vi "Generer_profil EPC3000.vi"(0 "Temps (s)":dbl[](array[numeric]) format="%#.1f", 1 "Num_Prog":u8, 2 "Températures (°C)":dbl[](array[numeric]) format="%#.1f", 3 "Evennements_entrée":T1, 4 "Programmes et config":T2 {"Programme 10"."Received Value" format="%#.1f"; "Programme 9"."Received Value" format="%#.1f"; "Programme 8"."Received Value" format="%#.1f"; "Programme 7"."Received Value" format="%#.1f"; "Programme 6"."Received Value" format="%#.1f"; "Programme 5"."Received Value" format="%#.1f"; "Configuration"."?" format="%#.1f"; "Programme 1"."Received Value" format="%#.1f"; "Programme 2"."Received Value" format="%#.1f"; "Programme 3"."Received Value" format="%#.1f"; "Programme 4"."Received Value" format="%#.1f"}) -> (5 "Temps (s)":dbl[](array[numeric]) format="%#.1f", 6 "Températures (°C)":dbl[](array[numeric]) format="%#.1f", 7 "Evennements_sortie":T1)   [LabVIEW 2022 SP3]
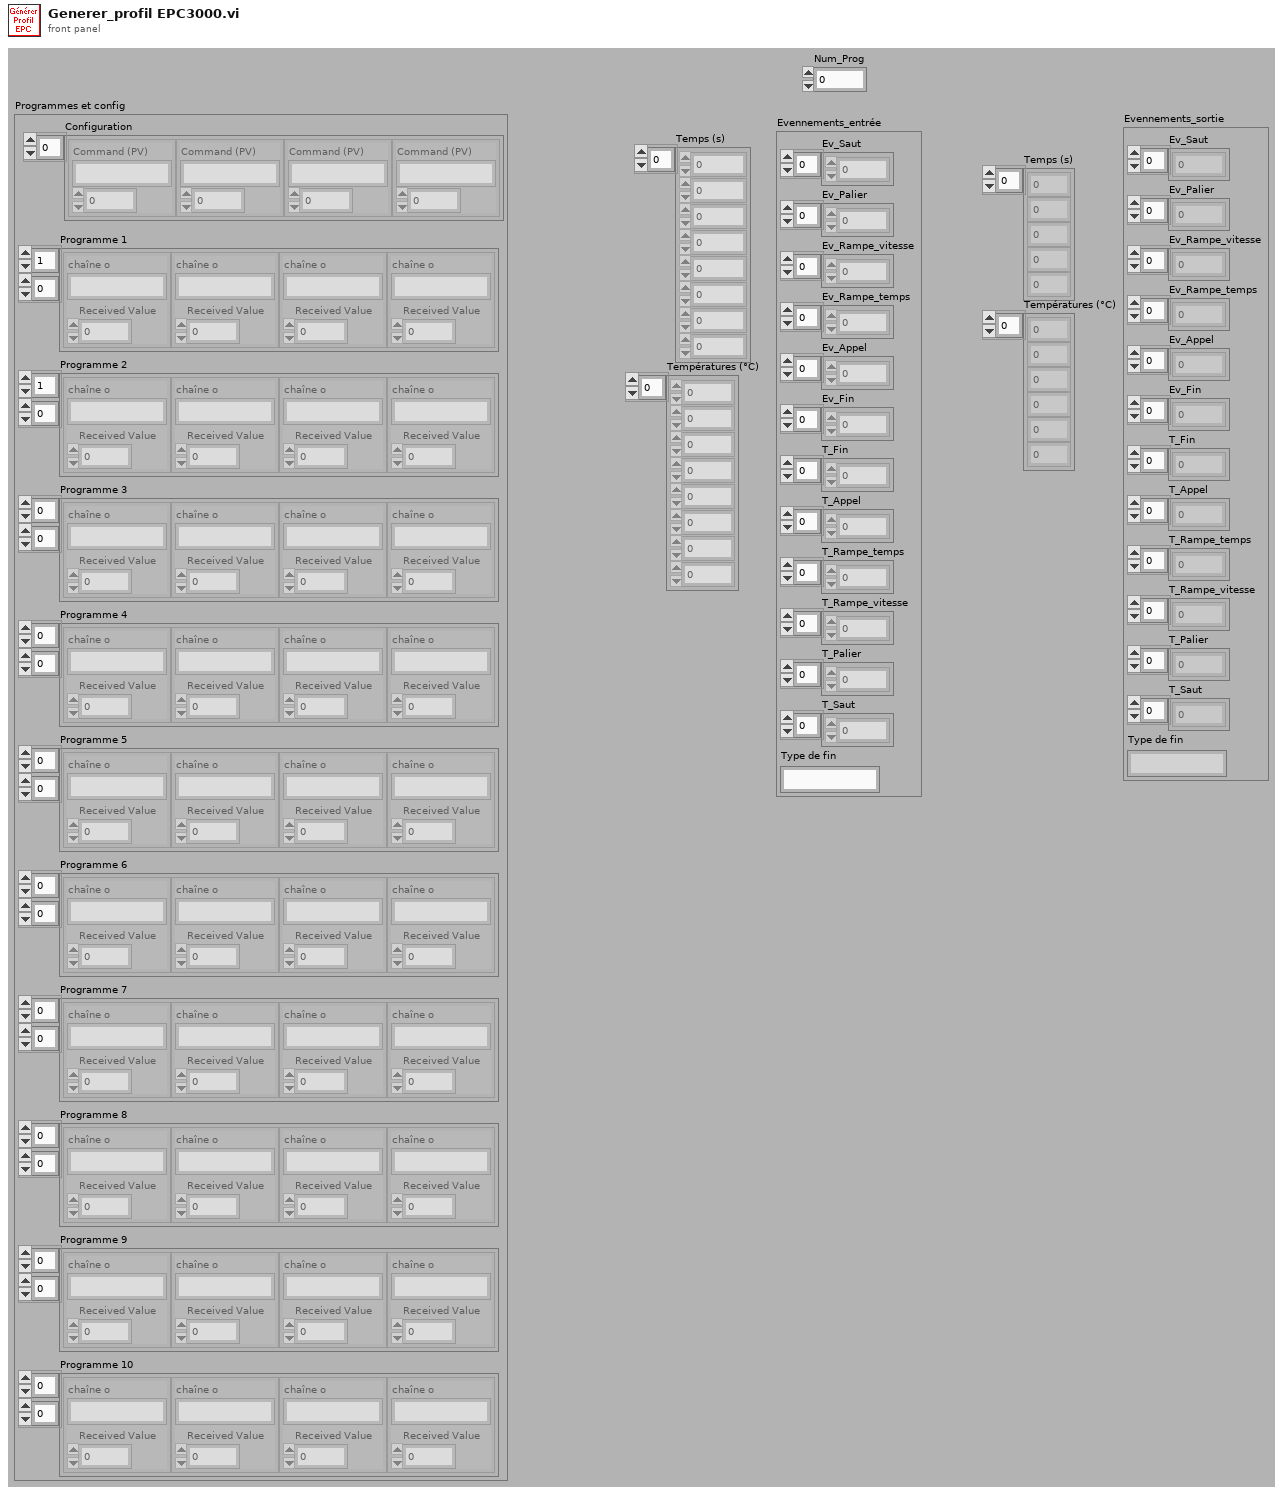
[diagram p1: front panel]
types:
  T1 = cluster{"Ev_Saut":dbl[], "Ev_Palier":dbl[], "Ev_Rampe_vitesse":dbl[], "Ev_Rampe_temps":dbl[], "Ev_Appel":dbl[], "Ev_Fin":dbl[], "T_Fin":dbl[], "T_Appel":dbl[], "T_Rampe_temps":dbl[], "T_Rampe_vitesse":dbl[], "T_Palier":dbl[], "T_Saut":dbl[], "Type de fin":string}
  T2 = cluster{"Configuration":cluster{"Command (PV)":string, dbl}[], "Programme 1":cluster{"chaîne o":string, "Received Value":dbl}[][], "Programme 2":cluster{"chaîne o":string, "Received Value":dbl}[][], "Programme 3":cluster{"chaîne o":string, "Received Value":dbl}[][], "Programme 4":cluster{"chaîne o":string, "Received Value":dbl}[][], "Programme 5":cluster{"chaîne o":string, "Received Value":dbl}[][], "Programme 6":cluster{"chaîne o":string, "Received Value":dbl}[][], "Programme 7":cluster{"chaîne o":string, "Received Value":dbl}[][], "Programme 8":cluster{"chaîne o":string, "Received Value":dbl}[][], "Programme 9":cluster{"chaîne o":string, "Received Value":dbl}[][], "Programme 10":cluster{"chaîne o":string, "Received Value":dbl}[][]}
  T3 = cluster{"chaîne o":string, "Received Value":dbl}[][]
  T4 = cluster{"chaîne o":string, "Received Value":dbl}[]
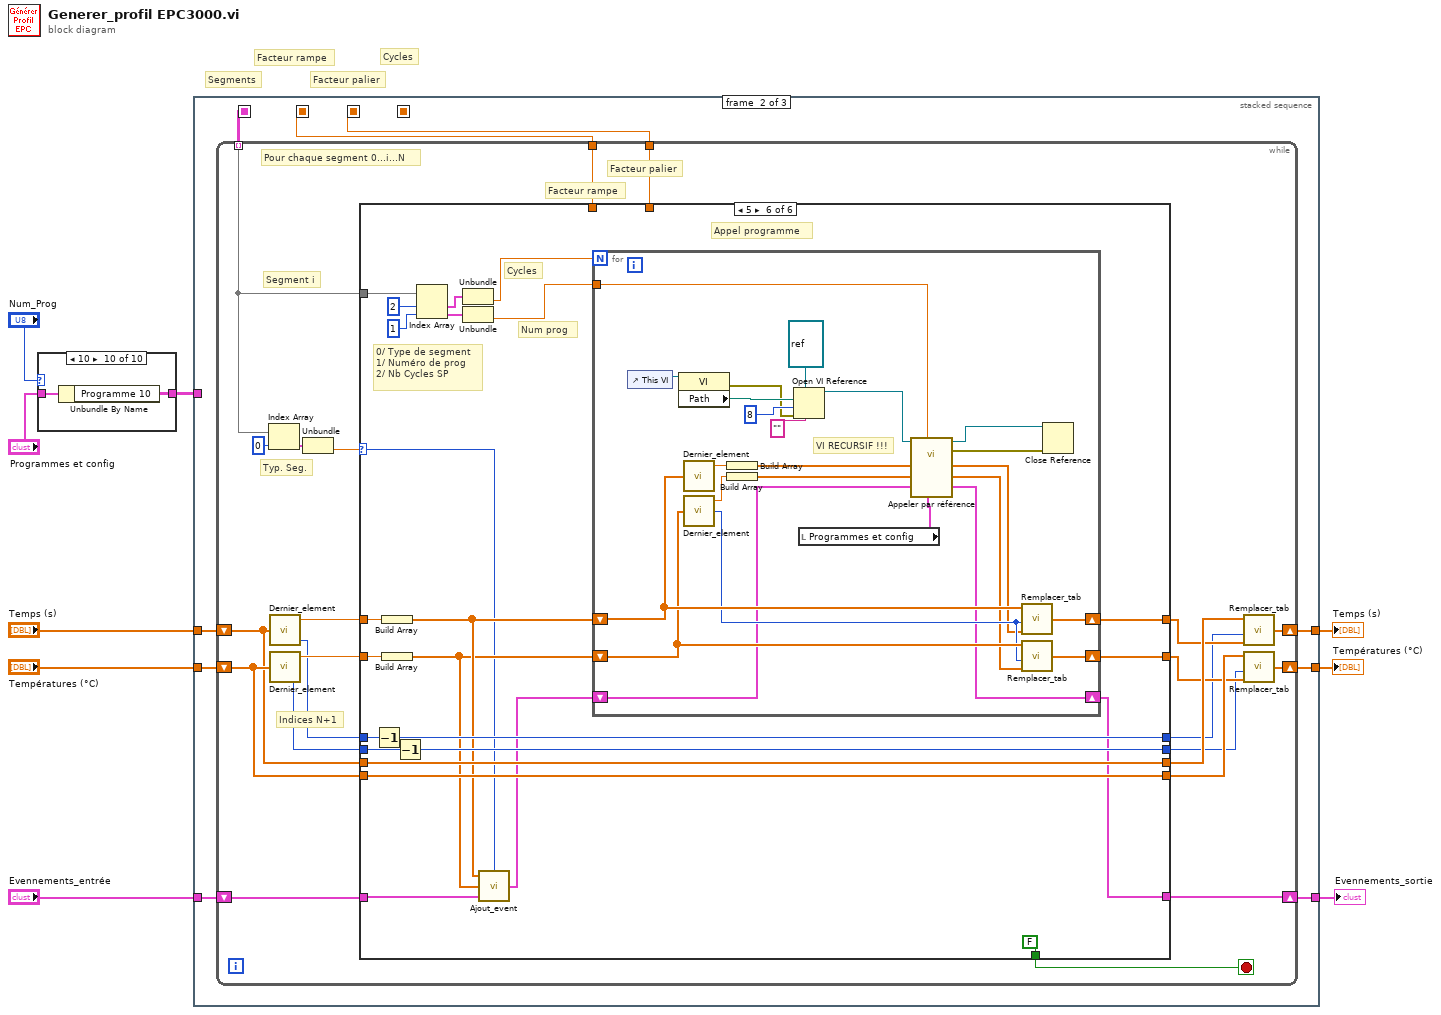
[diagram p0: block diagram]
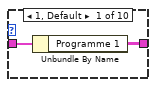
[diagram p2: hidden frame]
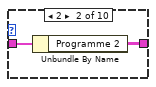
[diagram p3: hidden frame]
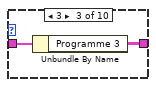
[diagram p4: hidden frame]
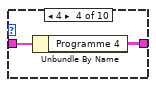
[diagram p5: hidden frame]
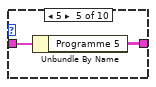
[diagram p6: hidden frame]
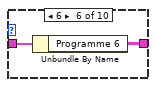
[diagram p7: hidden frame]
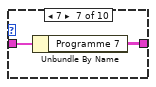
[diagram p8: hidden frame]
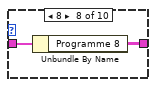
[diagram p9: hidden frame]
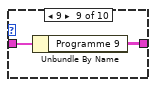
[diagram p10: hidden frame]
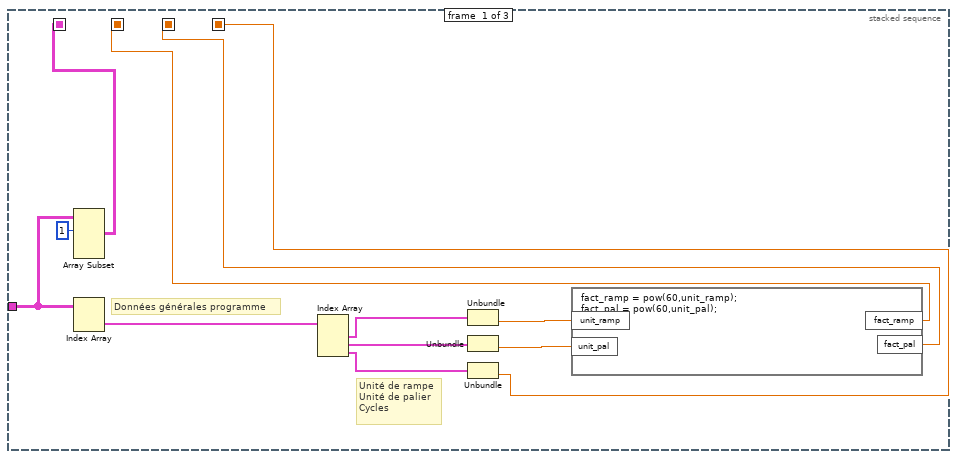
[diagram p11: hidden frame]
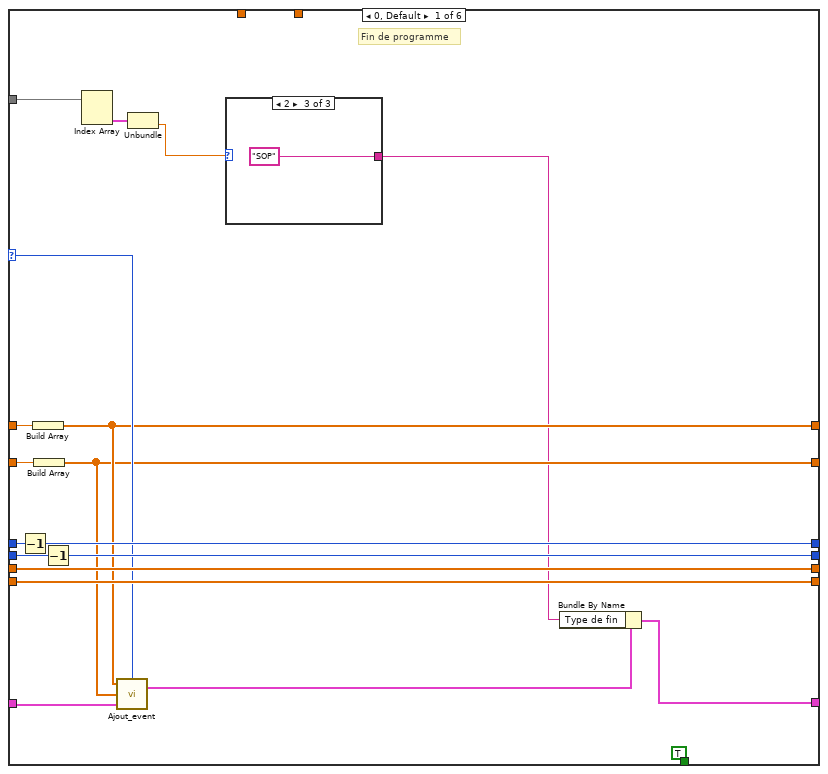
[diagram p12: hidden frame]
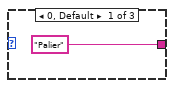
[diagram p13: hidden frame]
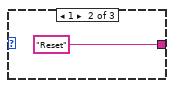
[diagram p14: hidden frame]
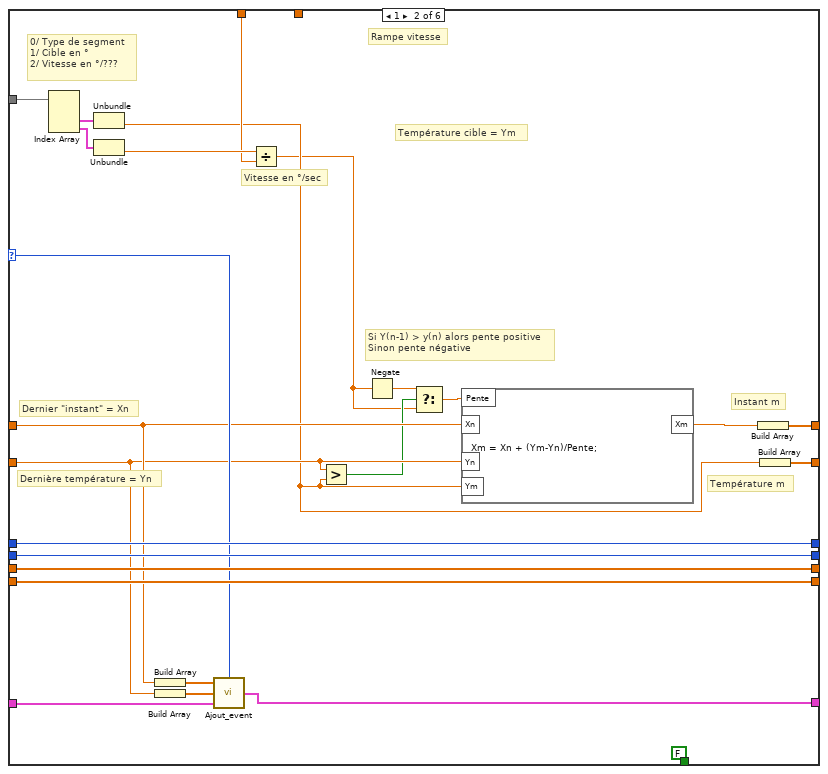
[diagram p15: hidden frame]
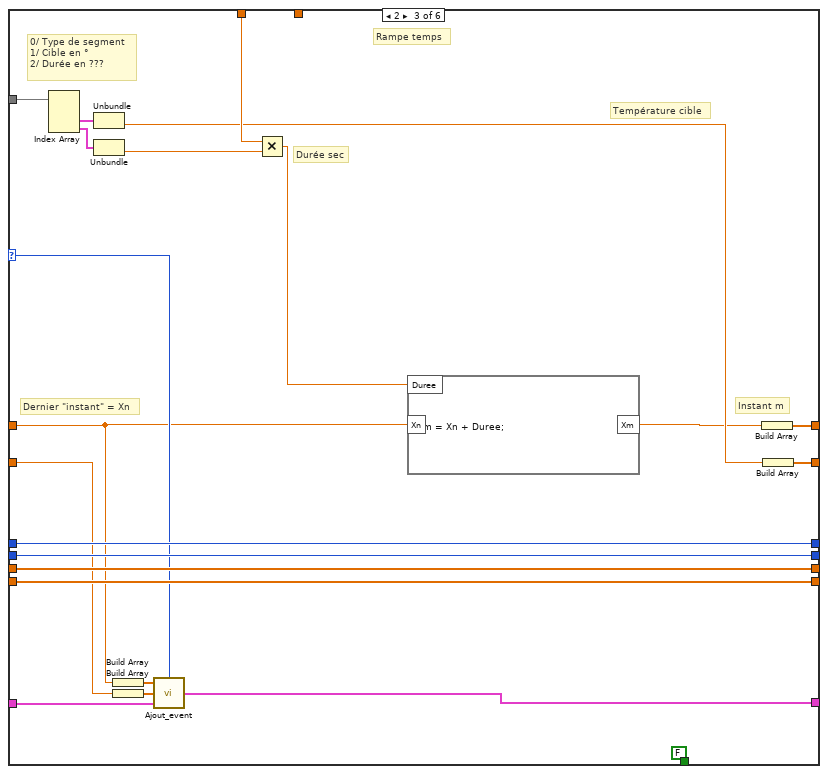
[diagram p16: hidden frame]
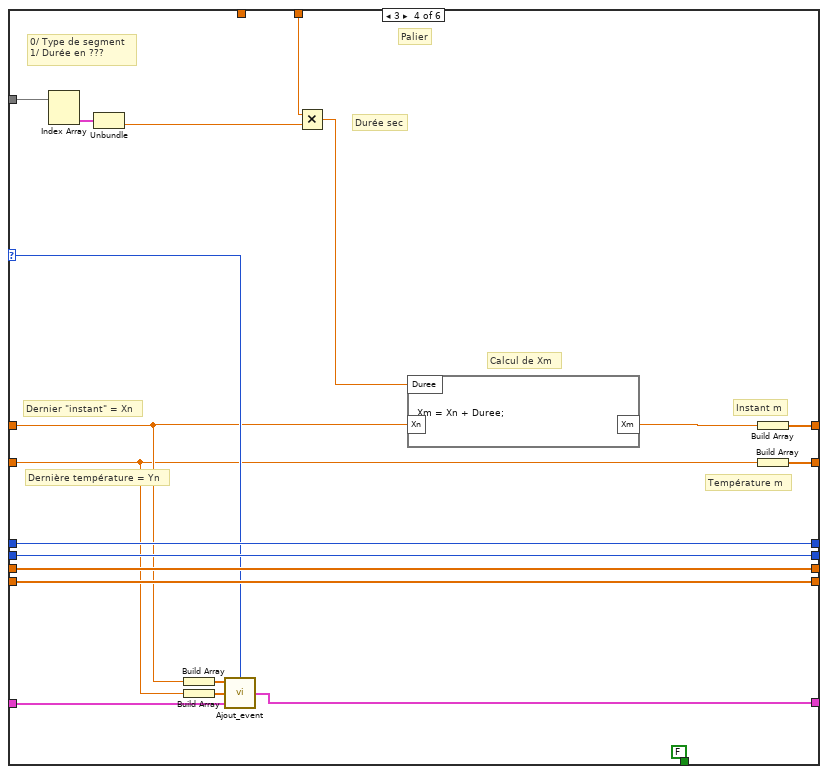
[diagram p17: hidden frame]
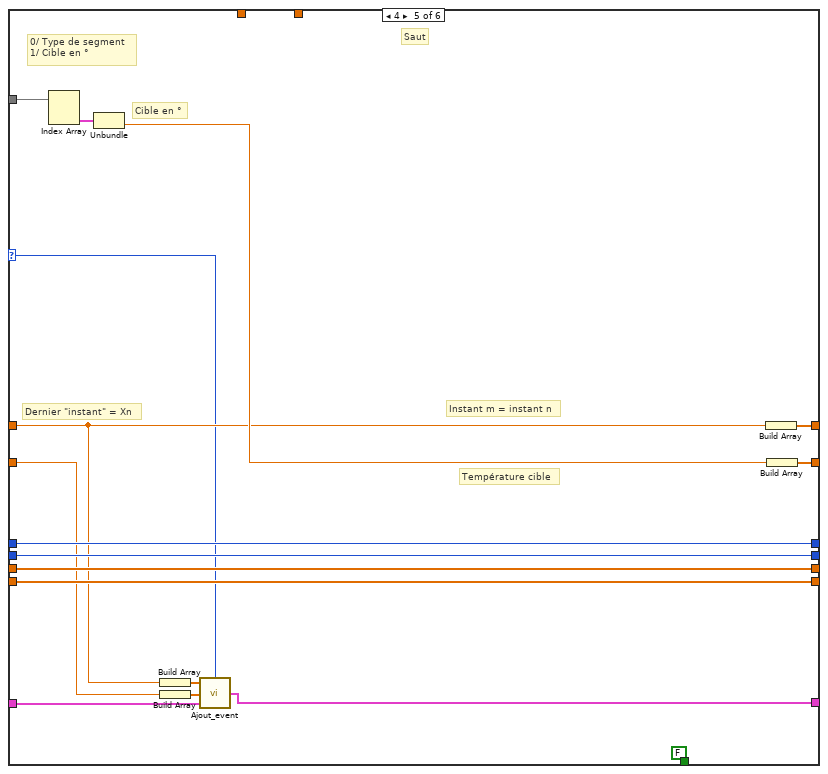
[diagram p18: hidden frame]
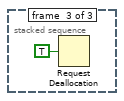
[diagram p19: hidden frame]
diagram:
  # "Facteur palier"
  # "Segments"
  # "Cycles"
  # "Facteur rampe"
  n1 = case shown="10" "Num_Prog" {
    tunnel: [w11 w13 w15 w17 w19 w21 w23 w25 w27 w29] -> w8
    tunnel: "Programmes et config" -> [w10 w12 w14 w16 w18 w20 w22 w24 w26 w28]
    frame 1, Default {
      n2 = Unbundle By Name(w10) -> ("Programme 1"=w11:T3)
    }
    frame 2 {
      n3 = Unbundle By Name(w12) -> ("Programme 2"=w13:T3)
    }
    frame 3 {
      n4 = Unbundle By Name(w14) -> ("Programme 3"=w15:T3)
    }
    frame 4 {
      n5 = Unbundle By Name(w16) -> ("Programme 4"=w17:T3)
    }
    frame 5 {
      n6 = Unbundle By Name(w18) -> ("Programme 5"=w19:T3)
    }
    frame 6 {
      n7 = Unbundle By Name(w20) -> ("Programme 6"=w21:T3)
    }
    frame 7 {
      n8 = Unbundle By Name(w22) -> ("Programme 7"=w23:T3)
    }
    frame 8 {
      n9 = Unbundle By Name(w24) -> ("Programme 8"=w25:T3)
    }
    frame 9 {
      n10 = Unbundle By Name(w26) -> ("Programme 9"=w27:T3)
    }
    frame 10 {
      n11 = Unbundle By Name(w28) -> ("Programme 10"=w29:T3)
    }
  }
  n12 = stacked-sequence {
    seq-local: [w31 _ _] -> [_ w50 _]
    seq-local: [w39 _ _] -> [_ w49 _]
    seq-local: [w38 _ _] -> [_ w48 _]
    seq-local: [w30 _ _] -> [_ _ _]
    tunnel: w8 -> [w36 _ _]
    tunnel: [_ w44 _] -> w4
    tunnel: [_ w45 _] -> w3
    tunnel: "Temps (s)" -> [_ w47 _]
    tunnel: "Températures (°C)" -> [_ w46 _]
    tunnel: "Evennements_entrée" -> [_ w43 _]
    tunnel: [_ w42 _] -> w1
    frame #0 {
      # "Données générales programme"
      # "Unité de rampe\nUnité de palier\nCycles"
      n13 = Array Subset(array=w36, index (row)=1 ("indice")) -> (w31:T3)  [unwired: 3 in]
      n14 = Index Array(array=w36) -> (element=w35:T4)  [unwired: 2 in]
      n15 = Index Array(array=w35) -> (element #1=w34:cluster{"chaîne o":string, "Received Value":dbl}, element #2=w33:cluster{"chaîne o":string, "Received Value":dbl}, element #3=w32:cluster{"chaîne o":string, "Received Value":dbl})  [unwired: 3 in]
      n16 = Unbundle(w34) -> ("Received Value"=w40:dbl)  [unwired: 1 out]
      n17 = Unbundle(w33) -> ("Received Value"=w41:dbl)  [unwired: 1 out]
      n18 = Unbundle(w32) -> ("Received Value"=w30:dbl)  [unwired: 1 out]
      n19 = formula code="fact_ramp = pow(60,unit_ramp);\nfact_pal = pow(60,unit_pal);"("unit_ramp"=w40, "unit_pal"=w41) -> ("fact_ramp"=w39:dbl, "fact_pal"=w38:dbl)
    }
    frame #1 {
      n20 = while {
        tunnel: w50 -> [w71] mode=indexing
        tunnel: w49 -> [w70]
        tunnel: w48 -> [w69]
        shift-right: [w59] -> w44
        shift-left: w47 -> [w61]
        shift-right: [w60] -> w45
        shift-left: w46 -> [w62]
        shift-right: [w51] -> w42
        shift-left: w43 -> [w52]
        stop <- w68 stop-if-true
        # "Indices N+1"
        # "Segment i"
        # "Facteur palier"
        # "Pour chaque segment 0...i...N"
        # "Facteur rampe"
        # "Typ. Seg."
        n21 = Index Array(array=w71, index=0 ("indice")) -> (element=w73:cluster{"chaîne o":string, "Received Value":dbl})
        n22 = call "Dernier_element.vi"("Tableau en entrée"=w61) -> ("Dernier élément"=w66:dbl, "Taille/Indice N+1"=w64:i32)  [unwired: 1 out]
        n23 = call "Dernier_element.vi"("Tableau en entrée"=w62) -> ("Dernier élément"=w65:dbl, "Taille/Indice N+1"=w63:i32)  [unwired: 1 out]
        n24 = Unbundle(w73) -> ("Received Value"=w67:dbl)  [unwired: 1 out]
        n25 = case shown="5" w67 {
          selector: w67 -> [w82 w107 w125 w147 w163 w180]
          tunnel: w71 -> [w78 w120 w142 w162 w179 w203]
          tunnel: w70 -> [_ w102 w138 _ _ _]
          tunnel: [w80 w117 w136 w155 w176 w192] -> w55
          tunnel: [w81 w116 w134 w157 w177 w193] -> w56
          tunnel: w66 -> [w91 w104 w124 w146 w167 w195]
          tunnel: w65 -> [w90 w101 w123 w144 w166 w194]
          tunnel: w69 -> [_ _ _ w158 _ _]
          tunnel: [TRUE FALSE FALSE FALSE FALSE FALSE] -> w68
          tunnel: w64 -> [w87 w113 w131 w153 w173 w191]
          tunnel: [w85 w113 w131 w153 w173 w188] -> w53
          tunnel: w63 -> [w86 w112 w130 w152 w172 w190]
          tunnel: [w84 w112 w130 w152 w172 w189] -> w54
          tunnel: w61 -> [w89 w111 w129 w151 w171 w187]
          tunnel: [w89 w111 w129 w151 w171 w187] -> w58
          tunnel: w62 -> [w88 w110 w128 w150 w170 w186]
          tunnel: [w88 w110 w128 w150 w170 w186] -> w57
          tunnel: w52 -> [w83 w109 w127 w149 w169 w185]
          tunnel: [w76 w108 w126 w148 w168 w181] -> w51
          frame 0, Default {
            # "Fin de programme"
            n26 = Decrement(x=w87) -> (x-1=w85:i32)
            n27 = Build Array(w91) -> (w81:dbl[])
            n28 = Build Array(w90) -> (w80:dbl[])
            n29 = Decrement(x=w86) -> (x-1=w84:i32)
            n30 = Index Array(array=w78) -> (element #2=w79:cluster{"chaîne o":string, "Received Value":dbl})  [unwired: 2 in, 1 out]
            n31 = call "Ajout_event.vi"("Type de segment"=w82, "Evennements_entrée"=w83, "Température"=w80, "Instant"=w81) -> ("Evennements_sortie"=w75:T1)
            n32 = Unbundle(w79) -> ("Received Value"=w77:dbl)  [unwired: 1 out]
            n33 = case shown="2" w77 {
              tunnel: ["Palier" "Reset" "SOP"] -> w74
              frame 0, Default {
              }
              frame 1 {
              }
              frame 2 {
              }
            }
            n34 = Bundle By Name(cluster=w75, "Type de fin"=w74) -> (w76:T1)
          }
          frame 1 {
            # "Si Y(n-1) > y(n) alors pente positive\nSinon pente négative"
            # "Température m"
            # "Instant m"
            # "Dernière température = Yn"
            # "Dernier \"instant\" = Xn"
            # "Calcul de Xm"
            # "Température cible = Ym"
            # "Vitesse en °/sec"
            # "0/ Type de segment\n1/ Cible en °\n2/ Vitesse en °/???"
            # "Rampe vitesse"
            n35 = Index Array(array=w120) -> (element #2=w119:cluster{"chaîne o":string, "Received Value":dbl}, element #3=w118:cluster{"chaîne o":string, "Received Value":dbl})  [unwired: 3 in, 1 out]
            n36 = Unbundle(w119) -> ("Received Value"=w100:dbl)  [unwired: 1 out]
            n37 = Unbundle(w118) -> ("Received Value"=w103:dbl)  [unwired: 1 out]
            n38 = Build Array(w104) -> (w106:dbl[])
            n39 = Build Array(w101) -> (w105:dbl[])
            n40 = call "Ajout_event.vi"("Type de segment"=w107, "Evennements_entrée"=w109, "Température"=w105, "Instant"=w106) -> ("Evennements_sortie"=w108:T1)
            n41 = Divide(x=w103, y=w102) -> (x/y=w96:dbl)
            n42 = Greater?(x=w101, y=w100) -> (0:w99:bool)
            n43 = Negate(x=w96) -> (-x=w97:dbl)
            n44 = Select(t=w97, s=w99, f=w96) -> (s? t:f=w98:dbl)
            n45 = formula code="Xm = Xn + (Ym-Yn)/Pente;"("Xn"=w104, "Yn"=w101, "Ym"=w100, "Pente"=w98) -> ("Xm"=w115:dbl)
            n46 = Build Array(w115) -> (w116:dbl[])
            n47 = Build Array(w100) -> (w117:dbl[])
          }
          frame 2 {
            # "Rampe temps"
            # "Température cible"
            # "Instant m"
            # "Dernier \"instant\" = Xn"
            # "Calcul de Xm"
            # "Durée sec"
            # "0/ Type de segment\n1/ Cible en °\n2/ Durée en ???"
            n48 = Index Array(array=w142) -> (element #2=w141:cluster{"chaîne o":string, "Received Value":dbl}, element #3=w140:cluster{"chaîne o":string, "Received Value":dbl})  [unwired: 3 in, 1 out]
            n49 = Unbundle(w141) -> ("Received Value"=w135:dbl)  [unwired: 1 out]
            n50 = Unbundle(w140) -> ("Received Value"=w139:dbl)  [unwired: 1 out]
            n51 = Build Array(w124) -> (w122:dbl[])
            n52 = Build Array(w123) -> (w121:dbl[])
            n53 = call "Ajout_event.vi"("Type de segment"=w125, "Evennements_entrée"=w127, "Température"=w121, "Instant"=w122) -> ("Evennements_sortie"=w126:T1)
            n54 = Multiply(x=w138, y=w139) -> (x*y=w137:dbl)
            n55 = formula code="Xm = Xn + Duree;"("Xn"=w124, "Duree"=w137) -> ("Xm"=w133:dbl)
            n56 = Build Array(w133) -> (w134:dbl[])
            n57 = Build Array(w135) -> (w136:dbl[])
          }
          frame 3 {
            # "Palier"
            # "Température m"
            # "Instant m"
            # "Dernière température = Yn"
            # "Dernier \"instant\" = Xn"
            # "Calcul de Xm"
            # "Durée sec"
            # "0/ Type de segment\n1/ Durée en ???"
            n58 = Index Array(array=w162) -> (element #2=w161:cluster{"chaîne o":string, "Received Value":dbl})  [unwired: 2 in, 1 out]
            n59 = Unbundle(w161) -> ("Received Value"=w159:dbl)  [unwired: 1 out]
            n60 = Build Array(w146) -> (w143:dbl[])
            n61 = Build Array(w144) -> (w145:dbl[])
            n62 = call "Ajout_event.vi"("Type de segment"=w147, "Evennements_entrée"=w149, "Température"=w145, "Instant"=w143) -> ("Evennements_sortie"=w148:T1)
            n63 = Multiply(x=w158, y=w159) -> (x*y=w160:dbl)
            n64 = formula code="Xm = Xn + Duree;"("Xn"=w146, "Duree"=w160) -> ("Xm"=w156:dbl)
            n65 = Build Array(w156) -> (w157:dbl[])
            n66 = Build Array(w144) -> (w155:dbl[])
          }
          frame 4 {
            # "Saut"
            # "Température cible"
            # "Instant m = instant n"
            # "Dernier \"instant\" = Xn"
            # "Cible en °"
            # "0/ Type de segment\n1/ Cible en °"
            n67 = Index Array(array=w179) -> (element #2=w178:cluster{"chaîne o":string, "Received Value":dbl})  [unwired: 2 in, 1 out]
            n68 = Unbundle(w178) -> ("Received Value"=w175:dbl)  [unwired: 1 out]
            n69 = Build Array(w167) -> (w165:dbl[])
            n70 = Build Array(w166) -> (w164:dbl[])
            n71 = call "Ajout_event.vi"("Type de segment"=w163, "Evennements_entrée"=w169, "Température"=w164, "Instant"=w165) -> ("Evennements_sortie"=w168:T1)
            n72 = Build Array(w167) -> (w177:dbl[])
            n73 = Build Array(w175) -> (w176:dbl[])
          }
          frame 5 {
            # "Cycles"
            # "Appel programme"
            # "Num prog"
            # "0/ Type de segment\n1/ Numéro de prog\n2/ Nb Cycles SP"
            n74 = Decrement(x=w191) -> (x-1=w188:i32)
            n75 = Build Array(w195) -> (w184:dbl[])
            n76 = Build Array(w194) -> (w183:dbl[])
            n77 = Decrement(x=w190) -> (x-1=w189:i32)
            n78 = Index Array(array=w203, index #1=2 ("indice"), index #2=1 ("indice")) -> (element #1=w199:cluster{"chaîne o":string, "Received Value":dbl}, element #2=w196:cluster{"chaîne o":string, "Received Value":dbl})
            n79 = Unbundle(w199) -> ("Received Value"=w198:dbl)  [unwired: 1 out]
            n80 = Unbundle(w196) -> ("Received Value"=w197:dbl)  [unwired: 1 out]
            n81 = call "Ajout_event.vi"("Type de segment"=w180, "Evennements_entrée"=w185, "Température"=w183, "Instant"=w184) -> ("Evennements_sortie"=w182:T1)
            n82 = for {
              N: w198 -> [_]
              tunnel: w197 -> [w214]
              shift-right: [w221] -> w193
              shift-left: w184 -> [w219]
              shift-right: [w220] -> w192
              shift-left: w183 -> [w218]
              shift-right: [w208] -> w181
              shift-left: w182 -> [w209]
              # "VI RECURSIF !!!"
              n83 = control-ref of="This VI"() -> (w226:refnum<vi>)
              n84 = property class="VI"(reference=w226) -> (error out=w222:errorcluster, "Path"=w225:path)  [unwired: 1 in, 1 out]
              n85 = call "Dernier_element.vi"("Tableau en entrée"=w219) -> ("Dernier élément"=w217:dbl)  [unwired: 2 out]
              n86 = call "Dernier_element.vi"("Tableau en entrée"=w218) -> ("Dernier élément"=w216:dbl, "Indice N"=w215:i32)  [unwired: 1 out]
              n87 = Build Array(w217) -> (w213:dbl[])
              n88 = Build Array(w216) -> (w212:dbl[])
              n89 = Open VI Reference(type specifier VI Refnum (for type only)=refnum<vi> refnum ("spécificateur de type du refnum de VI (pour type seulement)"), vi path=w225, options=8, password ("")="" ("mot de passe (\"\")"), error in (no error)=w222) -> (vi reference=w204:refnum<vi>)  [unwired: 1 in, 1 out]
              n90 = local read "Programmes et config"() -> (w207:T2)
              n91 = call-by-ref "Appeler par référence"(reference=w204, "Temps (s)"=w213, "Num_Prog"=w214, "Températures (°C)"=w212, "Evennements_entrée"=w209, "Programmes et config"=w207) -> (reference out=w224:refnum<vi>, error out=w223:errorcluster, "Temps (s)"=w210:dbl[], "Températures (°C)"=w211:dbl[], "Evennements_sortie"=w208:T1)  [unwired: 1 in]
              n92 = call "Remplacer_tab.vi"("Nouvel élément/sous tableau"=w210, "A partir de"=w215, "Tableau"=w219) -> ("Tableau inséré/remplacé"=w221:dbl[])  [unwired: 1 in]
              n93 = call "Remplacer_tab.vi"("Nouvel élément/sous tableau"=w211, "A partir de"=w215, "Tableau"=w218) -> ("Tableau inséré/remplacé"=w220:dbl[])  [unwired: 1 in]
              n94 = Close Reference(reference=w224, error in (no error)=w223) -> ()  [unwired: 1 out]
            }
          }
        }
        n95 = call "Remplacer_tab.vi"("Nouvel élément/sous tableau"=w56, "A partir de"=w53, "Tableau"=w58) -> ("Tableau inséré/remplacé"=w59:dbl[])  [unwired: 1 in]
        n96 = call "Remplacer_tab.vi"("Nouvel élément/sous tableau"=w55, "A partir de"=w54, "Tableau"=w57) -> ("Tableau inséré/remplacé"=w60:dbl[])  [unwired: 1 in]
      }
    }
    frame #2 {
      n97 = Request Deallocation(TRUE ("flag")) -> ()
    }
  }
  "Temps (s)" <- w4
  "Températures (°C)" <- w3
  "Evennements_sortie" <- w1
